vi "Test-1.vi"() -> ()   [LabVIEW 2021]
panel:
  out "Array":i32[](array[numeric])
  out "Number":i32
  in  "Multicolumn Listbox":i32(listbox)
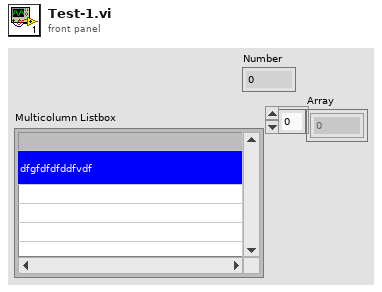
[diagram p1: front panel]
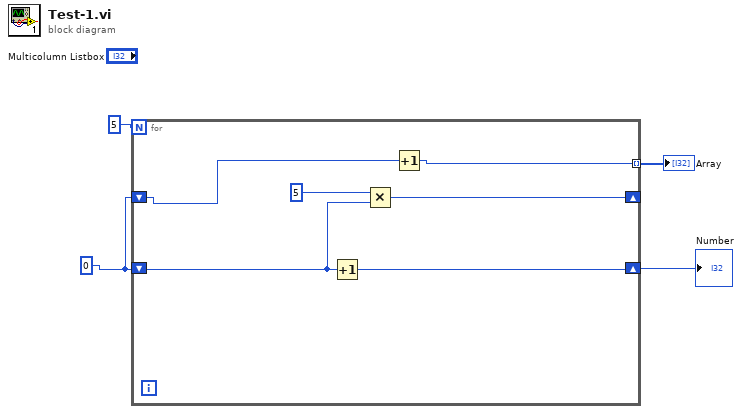
[diagram p0: block diagram]
diagram:
  w1 = 0
  n1 = for {
    N: 5 -> [_]
    shift-right: [w10] -> w3
    shift-left: w1 -> [w9]
    shift-right: [w7] -> _
    shift-left: w1 -> [w6]
    tunnel: [w5] -> w2 mode=indexing
    n2 = Increment(x=w9) -> (x+1=w10:i32)
    n3 = Multiply(x=5, y=w9) -> (x*y=w7:i32)
    n4 = Increment(x=w6) -> (x+1=w5:i32)
  }
  "Number" <- w3
  "Array" <- w2
